vi "AutoOp Default.vi"(10 "Occurrence Refnum":refnum<k4>, 11 "OpMode Index":u64 format="%.0x") -> ()   [LabVIEW 2023]
uses:
  <vilib>/MRC/Types/WPI_JoystickDeviceEnum.ctl
  <vilib>/MRC/MrcLib.lvlib
panel:
  out "Enabled":bool
  out "RobotMode":u8
  out "Match Time(s)":sgl
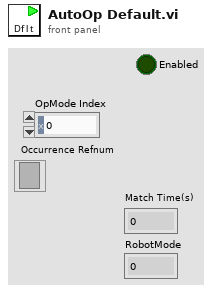
[diagram p1: front panel]
types:
  T1 = typedef "WPI_JoystickDeviceEnum.ctl" = enum16{"USB 0", "USB 1", "USB 2", "USB 3", "USB 4", "USB 5"}
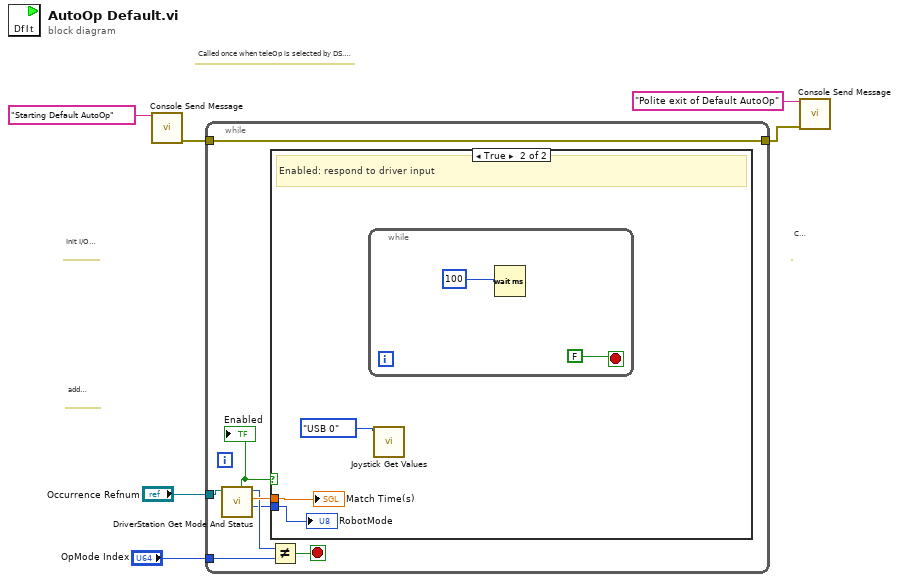
[diagram p0: block diagram]
diagram:
  # "add enabled counter\nstats, etc"
  # "Cleanup I/O"
  # "Called once when teleOp is selected by DS.\nLoop until mode changes carrying out enabled\nor disabled response."
  # "Init I/O and anything\nused during TeleOp"
  n1 = call <vilib>:"Console Send Message.vi"("Message"="Starting Default AutoOp") -> ("error out"=w4:errorcluster)  [unwired: 14 in]
  n2 = while {
    tunnel: "OpMode Index" -> [w13]
    tunnel: w4 -> [w9]
    tunnel: [w9] -> w2
    tunnel: "Occurrence Refnum" -> [w8]
    stop <- w12 stop-if-true
    n3 = call <vilib>:"DriverStation Get Mode And Status.vi"("Occurrence Refnum"=w8) -> ("RobotMode"=w10:u8, "Match Time(s)"=w14:sgl, "currentOpMode"=w11:u64, "Enabled"=w7:bool)  [unwired: 5 in, 2 out]
    "Enabled" <- w7
    n4 = Not Equal?(x=w11, y=w13) -> (x != y?=w12:bool)
    n5 = case shown="True" w7 {
      tunnel: w14 -> [_ w17]
      tunnel: w10 -> [_ w16]
      frame False {
        # "Disabled: update dashboard, possibly update state and setpoints for safer enable"
      }
      frame True {
        # "Enabled: respond to driver input"
        n6 = while {
          stop <- FALSE stop-if-true
          n7 = Wait (ms)(milliseconds to wait=u32 100) -> ()  [unwired: 1 out]
        }
        n8 = call <vilib>:"Joystick Get Values.vi"("Joystick"=WPI_JoystickDeviceEnum."USB 0") -> ()  [unwired: 5 in, 6 out]
        "Match Time(s)" <- w17
        "RobotMode" <- w16
      }
    }
  }
  n9 = call <vilib>:"Console Send Message.vi"("Message"="Polite exit of Default AutoOp", "error in (no error)"=w2) -> ()  [unwired: 13 in, 1 out]
